vi "CreateSimulated.vi"(8 "error in (no error)":errorcluster) -> (0 "error out":errorcluster, 3 "object out":refnum<class "AIO_Channel.lvclass">)   [LabVIEW 2021, in "Simulator-Channel.lvlib" / "AIO_Channel.lvclass"]
uses:
  AIO_Channel.lvclass
  AIO_Channel.lvclass/AIO_Channel.ctl
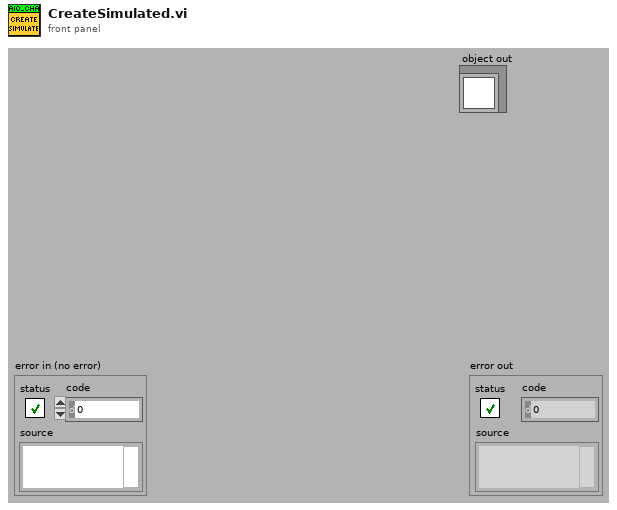
[diagram p1: front panel]
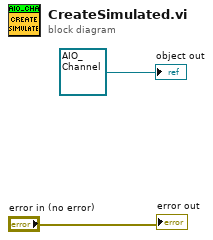
[diagram p0: block diagram]
diagram:
  "error out" <- "error in (no error)"
  "object out" <- refnum<class "AIO_Channel.lvclass"> refnum ("object in")
